vi "Render.vi"(8 "error in (no error)":errorcluster, 10 "String in":string, 11 "LinkingHeadingId in":refnum<class "LinkingHeadingId.lvclass">) -> (0 "error out":errorcluster, 2 "String out":string, 3 "LinkingHeadingId out":refnum<class "LinkingHeadingId.lvclass">)   [LabVIEW 2021, in "LvMarkdown.lvlib" / "LinkingHeadingId.lvclass"]
uses:
  LinkingHeadingId.lvclass
  C:/GitHub/LvMarkdown/src/LvMarkdown/Markdown.lvclass
  LinkingHeadingId.lvclass/LinkingHeadingId.ctl
  GetHeading.vi
  Heading/Heading.lvclass
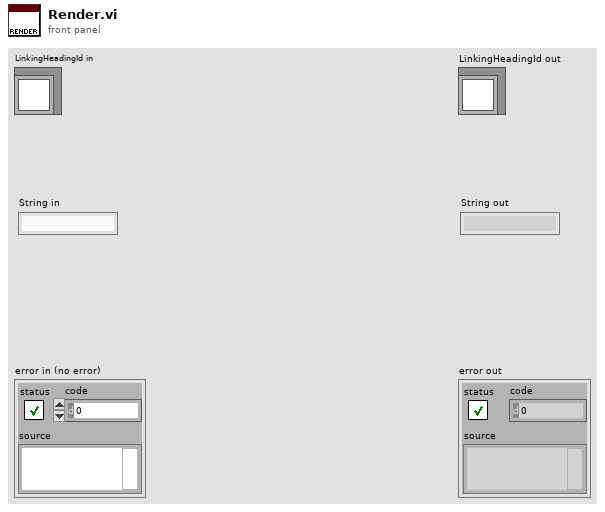
[diagram p1: front panel]
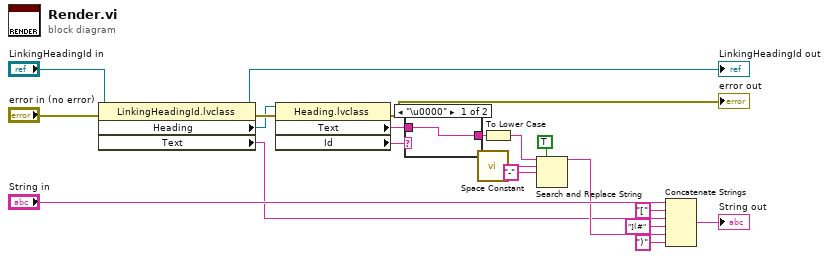
[diagram p0: block diagram]
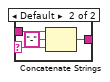
[diagram p2: hidden frame]
diagram:
  n1 = property class="LinkingHeadingId.lvclass"(reference="LinkingHeadingId in", error in="error in (no error)") -> (reference out=→"LinkingHeadingId out":refnum<class "LinkingHeadingId.lvclass">, error out=w13:errorcluster, "Heading"=w11:refnum<class "Heading.lvclass">, "Text"=w1:string)
  n2 = property class="Heading.lvclass"(reference=w11, error in=w13) -> (error out=→"error out":errorcluster, "Text"=w9:string, "Id"=w8:string)  [unwired: 1 out]
  n3 = case shown="\"\"" w8 {
    selector: w8 -> [_ w23]
    tunnel: w9 -> [w21 w25]
    tunnel: [w21 w22] -> w7
    frame "\u0000" {
    }
    frame Default {
      n4 = Concatenate Strings(w25, "-" ("string"), w23) -> (w22:string)
    }
  }
  n5 = call <vilib>:"Space Constant.vi"() -> ("String"=w5:string)
  n6 = To Lower Case(string=w7) -> (all lower case string=w6:string)
  n7 = Search and Replace String(replace all?=TRUE ("replace all? (F)"), input string=w6, search string=w5, replace string="-" ("replace string (\"\")")) -> (result string=w2:string)  [unwired: 4 in, 3 out]
  n8 = Concatenate Strings("String in", "[" ("string"), w1, "](#" ("string"), w2, ")" ("string")) -> (→"String out":string)
